vi "Is Available.vi"(8 "error in (no error)":errorcluster) -> (0 "error out":errorcluster, 3 "OUT":i32)   [LabVIEW 2011, in "HID_ARZ.lvlib"]
doc: "IS_AVAILABLE IsAvailable;"
uses:
  HID_ARZ.lvlib
  <userlib>/HID_ARZ/mcHID.dll
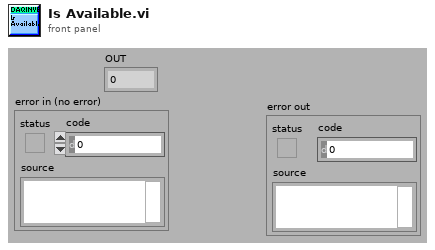
[diagram p1: front panel]
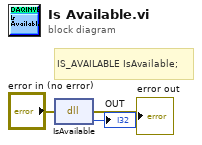
[diagram p0: block diagram]
diagram:
  # "IS_AVAILABLE IsAvailable;"
  n1 = dll-call lib="C:/Program Files (x86)/National Instruments/LabVIEW 2017/user.lib/HID_ARZ/mcHID.*" fn="IsAvailable"(error in="error in (no error)") -> (error out=→"error out":errorcluster, "return type"=→"OUT":i32)  [unwired: 2 in, 1 out]
